vi "VIH HelpGen - Build Named Numeric Ctrl Value Table.vi"(6 "Class":enum16{"Enum", "Ring"}(ring), 7 "EnumValDscr":T1[](array[typedef]), 9 "Table Template":string, 10 "Values":ext[](array[numeric]), 11 "Names":string[](array[string])) -> (2 "HTML out":string)   [LabVIEW 2014]
doc: "::: VI Helpeks :::\nCopyright (c) 2000-2026 Konstantin Shifershteyn. All rights reserved."
uses:
  VIH HelpGen Typedef - Cluster - Enum Value Info.ctl
panel:
  # "VI Helpeks\nCopyright (c) 2012-2026 Konstantin Shifershteyn"
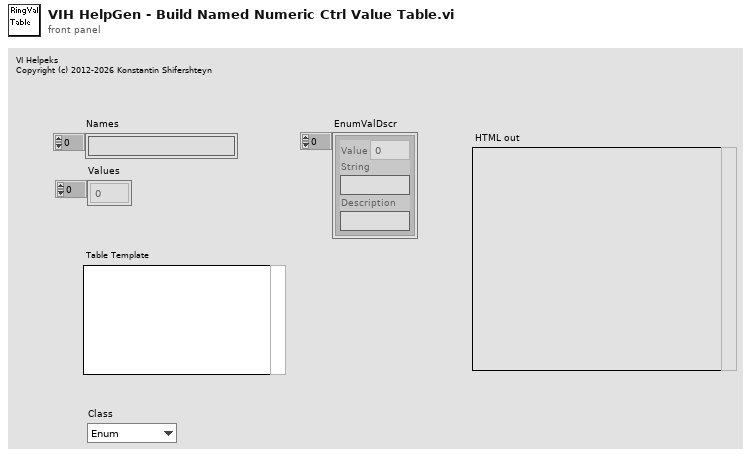
[diagram p1: front panel]
types:
  T1 = typedef "VIH HelpGen Typedef - Cluster - Enum Value Info.ctl" = cluster{"Value":ext, "String":string, "Description":string}
  T2 = enum16{"none", "LV description", "VH minimum", "VH extended"}
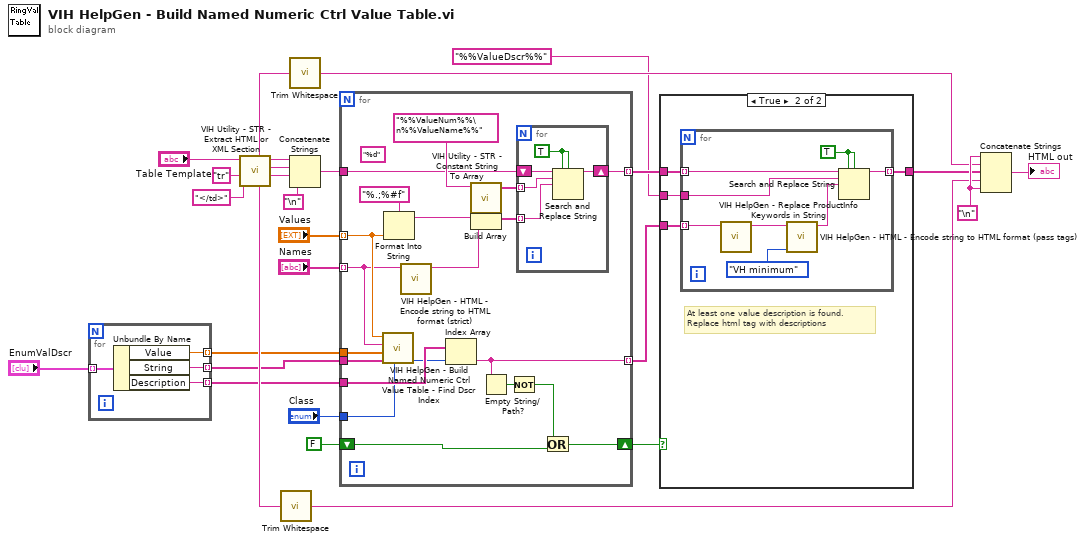
[diagram p0: block diagram]
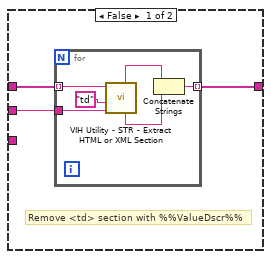
[diagram p2: hidden frame]
diagram:
  w19 = "\n"
  n1 = for {
    tunnel: "EnumValDscr" -> [w31] mode=indexing
    tunnel: [w30] -> w11 mode=indexing
    tunnel: [w29] -> w10 mode=indexing
    tunnel: [w28] -> w9 mode=indexing
    n2 = Unbundle By Name(w31) -> ("Value"=w30:ext, "String"=w29:string, "Description"=w28:string)
  }
  n3 = call "VIH Utility - STR - Extract HTML or XML Section.vi"("Contain (opt)"="</td>", "Section name"="tr", "HTML in"="Table Template") -> ("end"=w26:string, "body"=w25:string, "start"=w24:string, "after"=w18:string, "before"=w17:string)  [unwired: 4 in]
  n4 = call <vilib>:"Trim Whitespace.vi"("string"=w18) -> ("trimmed string"=w14:string)  [unwired: 1 in]
  n5 = call <vilib>:"Trim Whitespace.vi"("string"=w17) -> ("trimmed string"=w15:string)  [unwired: 1 in]
  n6 = Concatenate Strings(w24, w25, w26, "\n") -> (w6:string)
  n7 = for {
    tunnel: w6 -> [w48]
    tunnel: "Names" -> [w33] mode=indexing
    tunnel: "Values" -> [w44] mode=indexing
    tunnel: [w45] -> w4 mode=indexing
    tunnel: w11 -> [w43]
    tunnel: w10 -> [w42]
    tunnel: w9 -> [w41]
    tunnel: "Class" -> [w40]
    shift-right: [w38] -> w5
    shift-left: FALSE -> [w37]
    tunnel: [w36] -> w1 mode=indexing
    (unwired) "%d" ("format string")
    n8 = call "VIH HelpGen - Build Named Numeric Ctrl Value Table - Find Dscr Index.vi"("Class"=w40, "Strings"=w42, "Values"=w43, "String"=w33, "Value"=w44) -> ("Index"=w39:i32)  [unwired: 6 in]
    n9 = Format Into String(format string="%.;%#f", w44) -> (resulting string=w46:string)  [unwired: 2 in, 1 out]
    n10 = call "VIH HelpGen - HTML - Encode string to HTML format (strict).vi"("string"=w33) -> ("HTML string"=w32:string)  [unwired: 10 in]
    n11 = Index Array(array=w41, index=w39) -> (element=w36:string)
    n12 = call "VIH Utility - STR - Constant String To Array.vi"("String in"="%%ValueNum%%\n%%ValueName%%") -> ("Array out"=w50:string[])  [unwired: 10 in]
    n13 = Build Array(w46, w32) -> (w51:string[])
    n14 = Empty String/Path?(string/path=w36) -> (empty?=w35:bool)
    n15 = Not(x=w35) -> (.not. x?=w34:bool)
    n16 = for {
      shift-right: [w55] -> w45
      shift-left: w48 -> [w56]
      tunnel: w50 -> [w53] mode=indexing
      tunnel: w51 -> [w52] mode=indexing
      w54 = TRUE
      n17 = Search and Replace String(replace all?=w54, case sensitive?=w54, input string=w56, search string=w53, replace string=w52) -> (result string=w55:string)  [unwired: 3 in, 3 out]
    }
    n18 = Or(x=w34, y=w37) -> (x .or. y?=w38:bool)
  }
  n19 = case shown="True" w5 {
    tunnel: w4 -> [w59 w69]
    tunnel: [w58 w68] -> w3
    tunnel: "%%ValueDscr%%" ("search string/char (-)") -> [w57 w67]
    tunnel: w1 -> [_ w66]
    frame False {
      # "Remove <td> section with %%ValueDscr%%"
      n20 = for {
        tunnel: w59 -> [w64] mode=indexing
        tunnel: [w61] -> w58 mode=indexing
        tunnel: w57 -> [w60]
        n21 = call "VIH Utility - STR - Extract HTML or XML Section.vi"("Contain (opt)"=w60, "Section name"="td", "HTML in"=w64) -> ("after"=w62:string, "before"=w63:string)  [unwired: 4 in, 3 out]
        n22 = Concatenate Strings(w63, w62) -> (w61:string)
      }
    }
    frame True {
      # "At least one value description is found.\nReplace html tag with descriptions"
      n23 = for {
        tunnel: w69 -> [w77] mode=indexing
        tunnel: [w75] -> w68 mode=indexing
        tunnel: w67 -> [w74]
        tunnel: w66 -> [w71] mode=indexing
        w76 = TRUE
        n24 = call "VIH HelpGen - Replace ProductInfo Keywords in String.vi"("String in"=w71) -> ("String out"=w70:string)  [unwired: 10 in]
        n25 = call "VIH HelpGen - HTML - Encode string to HTML format (pass tags).vi"("HTML Tagset allowed"=T2."VH minimum" ("Tag set"), "string"=w70) -> ("HTML string"=w73:string)  [unwired: 9 in]
        n26 = Search and Replace String(replace all?=w76, case sensitive?=w76, input string=w77, search string=w74, replace string=w73) -> (result string=w75:string)  [unwired: 3 in, 3 out]
      }
    }
  }
  n27 = Concatenate Strings(w19, w15, w3, w14, w19) -> (→"HTML out":string)
